vi "[ce] CE component paths.vi"(0 "kind of path":T1, 1 "append path":string) -> (2 "path out":path)   [LabVIEW 2021]
doc: "::: CalcExpress Toolkit :::\nCopyright (c) 2000-2026 Konstantin Shifershteyn. All rights reserved."
uses:
  [ce] CE component paths - Kind of Path Enum.ctl
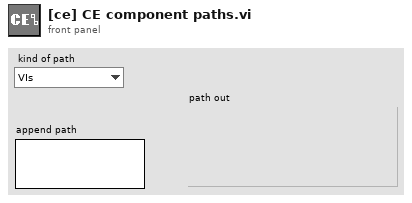
[diagram p1: front panel]
types:
  T1 = typedef "[ce] CE component paths - Kind of Path Enum.ctl" = enum16{"VIs", "FuncVIs", "Help", "Examples", "Project", "Templates"}
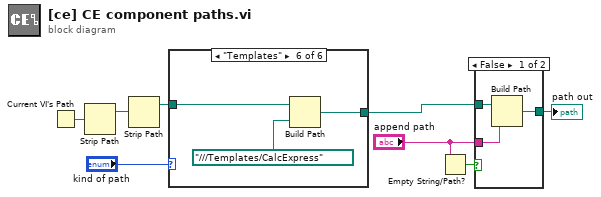
[diagram p0: block diagram]
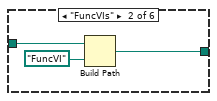
[diagram p4: hidden frame]
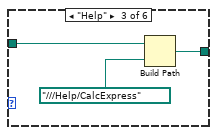
[diagram p5: hidden frame]
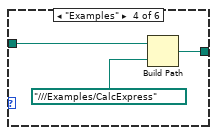
[diagram p6: hidden frame]
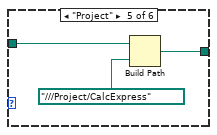
[diagram p7: hidden frame]
diagram:
  n1 = Current VI's Path() -> (path=w1:path)
  n2 = Strip Path(path=w1) -> (stripped path=w8:path)  [unwired: 1 out]
  n3 = Strip Path(path=w8) -> (stripped path=w6:path)  [unwired: 1 out]
  n4 = case shown="\"Templates\"" "kind of path" {
    tunnel: [w9 w10 w14 w16 w20 w23] -> w5
    tunnel: w6 -> [w9 w12 w15 w18 w21 w24]
    frame "VIs" {
    }
    frame "FuncVIs" {
      n5 = Build Path(base path=w12, name or relative path=path "FuncVI") -> (appended path=w10:path)
    }
    frame "Help" {
      n6 = Build Path(base path=w15, name or relative path=path "../../../Help/CalcExpress") -> (appended path=w14:path)
    }
    frame "Examples" {
      n7 = Build Path(base path=w18, name or relative path=path "../../../Examples/CalcExpress") -> (appended path=w16:path)
    }
    frame "Project" {
      n8 = Build Path(base path=w21, name or relative path=path "../../../Project/CalcExpress") -> (appended path=w20:path)
    }
    frame "Templates" {
      n9 = Build Path(base path=w24, name or relative path=path "../../../Templates/CalcExpress") -> (appended path=w23:path)
    }
  }
  n10 = Empty String/Path?(string/path="append path") -> (empty?=w3:bool)
  n11 = case shown="False" w3 {
    tunnel: w5 -> [w27 w28]
    tunnel: "append path" -> [w26 _]
    tunnel: [w25 w28] -> w2
    frame False {
      n12 = Build Path(base path=w27, name or relative path=w26) -> (appended path=w25:path)
    }
    frame True {
    }
  }
  "path out" <- w2
